vi "Write Image.vi"(8 "error in (no error)":errorcluster, 9 "Paths":path[](array[path]), 10 "ImageWriteBuffer":u16[](array[numeric]), 11 "ImageHandler:Varex-ImageHandler in":refnum<class "Varex-ImageHandler.lvclass">) -> (0 "error out":errorcluster, 3 "ImageHandler:Varex-ImageHandler out":refnum<class "Varex-ImageHandler.lvclass">)   [LabVIEW 2022 SP3, in "ImageHandler.lvlib" / "Varex-ImageHandler.lvclass"]
uses:
  Varex-ImageHandler.lvclass
  C:/Program Files/National Instruments/LabVIEW 2025/vi.lib/ActorFramework/Actor/Actor.lvclass
  Varex-ImageHandler.lvclass/Varex-ImageHandler.ctl
  <vilib>/ActorFramework/Actor/Actor.lvclass/Actor.ctl
  ImageHandler - Controller -- Interface/ImageHandler - Controller -- Interface Messages/Acquisition Status Msg/Acquisition Status Msg.lvclass/Acquisition Status Msg.ctl
  <vilib>/ActorFramework/Message Enqueuer/Message Enqueuer.lvclass/Message Enqueuer.ctl
  <vilib>/ActorFramework/Message Enqueuer/Enqueue.vi
  ImageHandler - Controller -- Interface/ImageHandler - Controller -- Interface Messages/Acquisition Status Msg/Acquisition Status Msg.lvclass
  C:/Program Files/National Instruments/LabVIEW 2025/vi.lib/ActorFramework/Message/Message.lvclass
  <vilib>/ActorFramework/Message Priority Queue/Priority Enqueue.vi
  <vilib>/ActorFramework/Actor/Actor.lvclass
panel:
  out "Time":u32
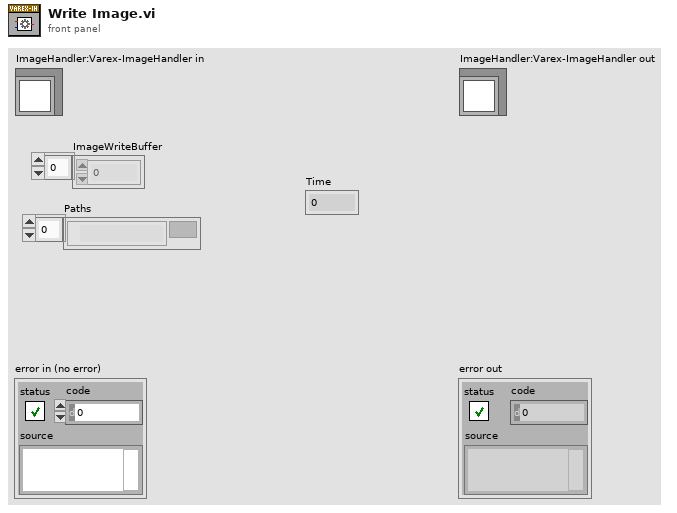
[diagram p1: front panel]
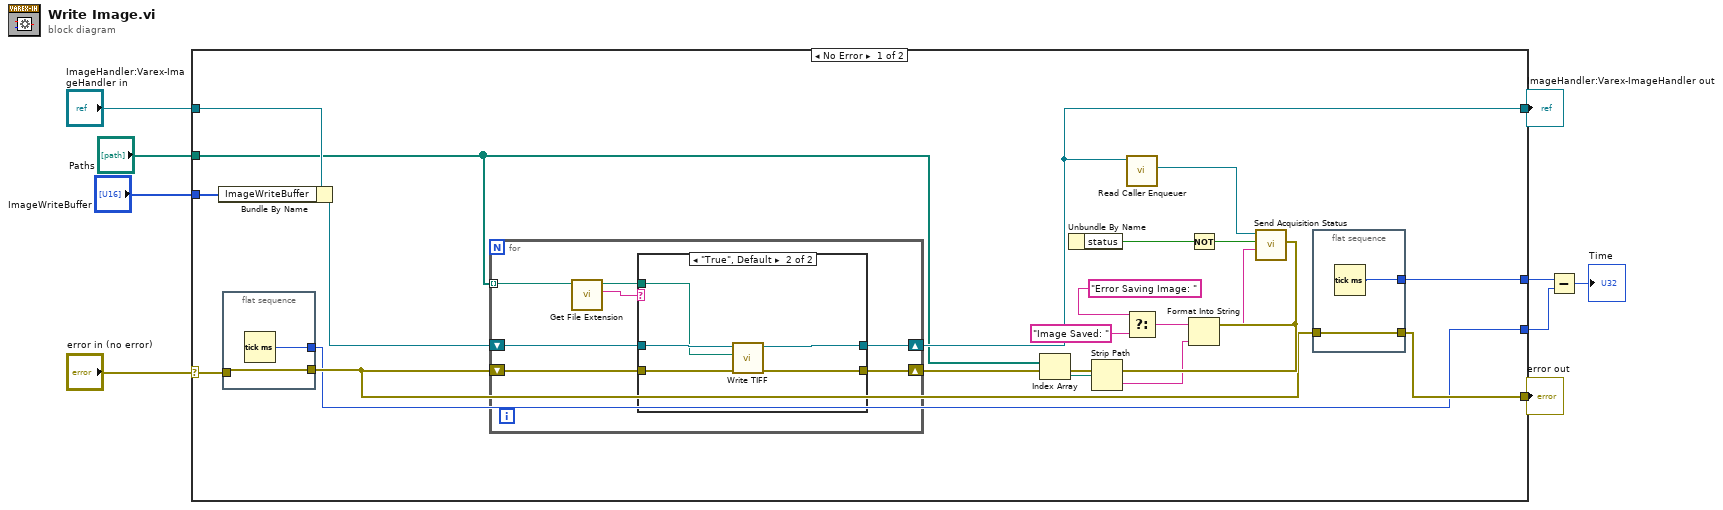
[diagram p0: block diagram]
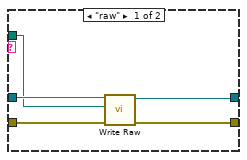
[diagram p2: hidden frame]
diagram:
  n1 = case shown="No Error" "error in (no error)" {
    selector: "error in (no error)" -> [w14 w52]
    tunnel: [w12 w52] -> w8
    tunnel: [w23 w51] -> w6
    tunnel: "ImageHandler:Varex-ImageHandler in" -> [w25 w51]
    tunnel: "Paths" -> [w15 _]
    tunnel: "ImageWriteBuffer" -> [w24 _]
    tunnel: [w11 _] -> w3
    tunnel: [w10 _] -> w2
    frame No Error {
      n2 = Bundle By Name(cluster=w25, "ImageWriteBuffer"=w24) -> (w26:refnum<class "Varex-ImageHandler.lvclass">)
      n3 = flat-sequence {
        tunnel: [w31] -> w10
        tunnel: w14 -> [w30]
        tunnel: [w30] -> w13
        frame #0 {
          n4 = Tick Count (ms)() -> (millisecond timer value=w31:u32)
        }
      }
      n5 = for {
        tunnel: w15 -> [w34] mode=indexing
        shift-right: [w39] -> w20
        shift-left: w13 -> [w38]
        shift-right: [w40] -> w23
        shift-left: w26 -> [w37]
        n6 = call <vilib>:"Get File Extension.vi"("file"=w34) -> ("lowercase file extension"=w35:string, "dup file"=w36:path)  [unwired: 6 in, 3 out]
        n7 = case shown="\"True\", Default" w35 {
          tunnel: w37 -> [w45 w50]
          tunnel: [w44 w49] -> w40
          tunnel: w38 -> [w43 w48]
          tunnel: [w42 w47] -> w39
          tunnel: w36 -> [w41 w46]
          frame "raw" {
            n8 = call-dynamic "Write Raw.vi"("error in (no error)"=w43, "Path"=w41, "ImageHandler:Varex-ImageHandler in"=w45) -> ("error out"=w42:errorcluster, "ImageHandler:Varex-ImageHandler out"=w44:refnum<class "Varex-ImageHandler.lvclass">)  [unwired: 7 in]
          }
          frame "True", Default {
            n9 = call-dynamic "Write TIFF.vi"("error in (no error)"=w48, "Path"=w46, "ImageHandler:Varex-ImageHandler in"=w50) -> ("error out"=w47:errorcluster, "ImageHandler:Varex-ImageHandler out"=w49:refnum<class "Varex-ImageHandler.lvclass">)  [unwired: 7 in]
          }
        }
      }
      n10 = Index Array(array=w15) -> (element=w19:path)  [unwired: 1 in]
      n11 = Unbundle By Name(w20) -> ("status"=w28:bool)
      n12 = Strip Path(path=w19) -> (name=w18:string)  [unwired: 1 out]
      n13 = call <vilib>:"Read Caller Enqueuer.vi"("Actor"=w23) -> ("Caller Enqueuer"=w29:refnum<class "Message Enqueuer.lvclass">)  [unwired: 10 in]
      n14 = Select(t="Error Saving Image: ", s=w20, f="Image Saved: ") -> (s? t:f=w22:string)
      n15 = Not(x=w28) -> (.not. x?=w27:bool)
      n16 = Format Into String(initial string=w22, w18) -> (resulting string=w17:string)  [unwired: 2 in, 1 out]
      n17 = call "Send Acquisition Status.vi"("Remarks"=w17, "Status"=w27, "Message Enqueuer"=w29) -> ()  [unwired: 7 in, 2 out]
      n18 = flat-sequence {
        tunnel: w13 -> [w33]
        tunnel: [w33] -> w12
        tunnel: [w32] -> w11
        frame #0 {
          n19 = Tick Count (ms)() -> (millisecond timer value=w32:u32)
        }
      }
    }
    frame Error {
    }
  }
  "error out" <- w8
  "ImageHandler:Varex-ImageHandler out" <- w6
  n20 = Subtract(x=w3, y=w2) -> (x-y=→"Time":u32)
